vi "InstallVIPMPackage.vi"(7 "labview version":string, 8 "error in":errorcluster, 11 "vipc file":path) -> (0 "error out":errorcluster)   [LabVIEW 2019]
uses:
  <vilib>/JKI/VIPM API/VIPM API_vipm_api.lvlib
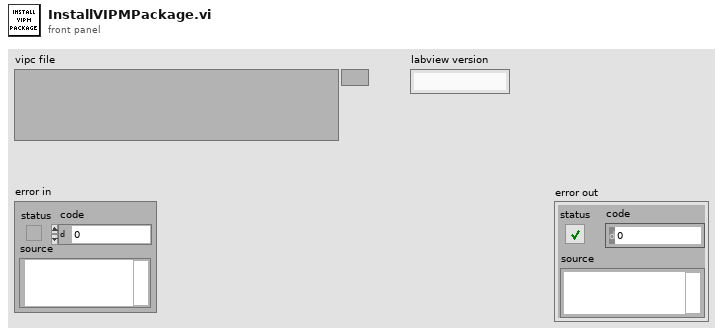
[diagram p1: front panel]
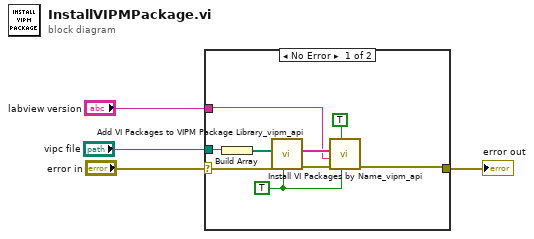
[diagram p0: block diagram]
diagram:
  n1 = case shown="No Error" "error in" {
    selector: "error in" -> [w11 w14]
    tunnel: [w6 w14] -> w3
    tunnel: "vipc file" -> [w13 _]
    tunnel: "labview version" -> [w5 _]
    frame No Error {
      w7 = TRUE ("quiet? (T)")
      n2 = Build Array(w13) -> (w12:path[])
      n3 = call <vilib>:"Add VI Packages to VIPM Package Library_vipm_api.vi"("quiet? (T)"=w7, "error in (no error)"=w11, "Packages to add to VIPM Library (vipc,vip,ogp)"=w12) -> ("error out"=w10:errorcluster, "Package Names Added"=w9:string[])  [unwired: 7 in]
      n4 = call <vilib>:"Install VI Packages by Name_vipm_api.vi"("quiet? (T)"=w7, "accept-eulas? (T)"=TRUE, "error in (no error)"=w10, "LabVIEW Version"=w5, "Package Names to Install []"=w9) -> ("error out"=w6:errorcluster)  [unwired: 6 in]
    }
    frame Error {
    }
  }
  "error out" <- w3
